vi "Init.vi"(8 "error in (no error)":errorcluster, 10 "ID":string, 11 "Deck in":refnum<class "Deck.lvclass">) -> (0 "error out":errorcluster, 3 "Deck out":refnum<class "Deck.lvclass">)   [LabVIEW 2019, in "Deck.lvclass"]
uses:
  Deck.lvclass
  State.ctl
  Packed Libraries/Audio Processing.lvlibp/Value Cluster.ctl
  Packed Libraries/Audio Processing.lvlibp/Value Properties.ctl
  Libraries/Track Info/Track Info.ctl
  Deck.lvclass/Deck.ctl
  Packed Libraries/Globals.lvlibp/Constants.vi
  Packed Libraries/Audio Processing.lvlibp
  Packed Libraries/Messaging.lvlibp
  Packed Libraries/Globals.lvlibp
  Libraries/Track Info/Track Info.lvlib
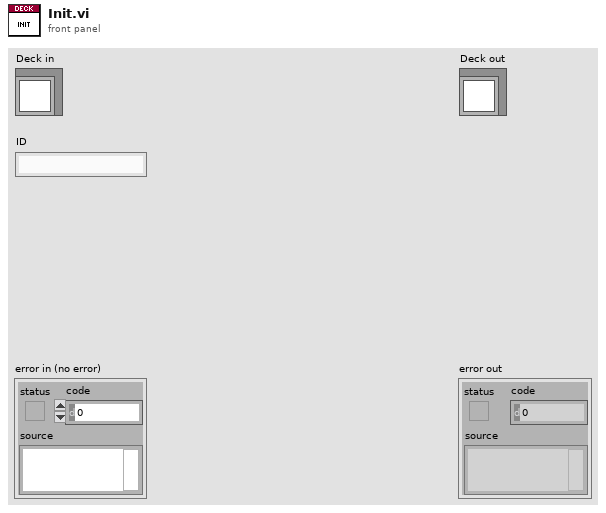
[diagram p1: front panel]
types:
  T1 = typedef "Track Info.lvlib/Track Info.ctl" = cluster{"Path":path, "Length (Samples)":i32, "Channels":i32, "Sample Rate (Hz)":i32, "BPM":dbl, "Cue Points (Samples)":i32[]}
  T2 = typedef "Audio Processing.lvlibp/Value Cluster.ctl" = cluster{"Value":dbl, "Properties":T3}
  T3 = typedef "Audio Processing.lvlibp/Value Properties.ctl" = cluster{"Lower":dbl, "Upper":dbl, "Default":dbl, "Increment":dbl}
  T4 = typedef "Deck.lvclass/State.ctl" = enum16{"No Track", "Loading", "Active", "Scratching", "Brake", "Backspin"}
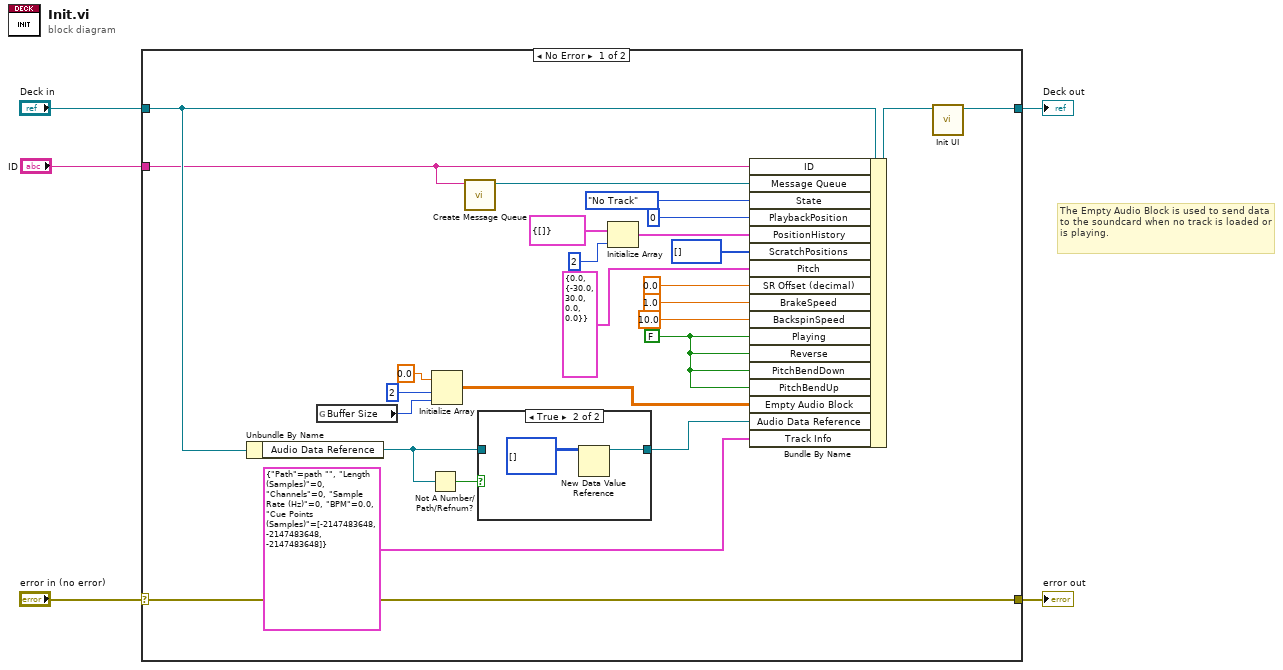
[diagram p0: block diagram]
diagram:
  # "The Empty Audio Block is used to send data to the soundcard when no track is loaded or is playing."
  n1 = case shown="No Error" "error in (no error)" {
    selector: "error in (no error)" -> [w30 w35]
    tunnel: [w30 w35] -> w4
    tunnel: [w6 w34] -> w2
    tunnel: "Deck in" -> [w25 w34]
    tunnel: "ID" -> [w12 _]
    frame No Error {
      w16 = FALSE ("PitchBendDown")
      n2 = Unbundle By Name(w25) -> ("Audio Data Reference"=w22:refnum<data-value>)
      n3 = global read "Constants.vi" "Buffer Size"() -> (w10:i32)
      n4 = Not A Number/Path/Refnum?(number/path/refnum=w22) -> (NaN/Path/Refnum?=w24:bool)
      n5 = Initialize Array(0.0, 2 ("dimension size"), w10) -> (w26:dbl[][])
      n6 = call "Create Message Queue.vi"("Queue Name"=w12) -> ("queue out"=w11:refnum<queue>)  [unwired: 9 in, 1 out]
      n7 = case shown="True" w24 {
        tunnel: [w31 w33] -> w23
        tunnel: w22 -> [w31 _]
        frame False {
        }
        frame True {
          n8 = New Data Value Reference(data value=i16[][] [] ("Audio Data")) -> (data value reference=w33:refnum<data-value>)  [unwired: 1 in, 1 out]
        }
      }
      n9 = Initialize Array(cluster{"Positions":i32[]} {"Positions"=[]} ("Cluster"), 2 ("dimension size")) -> (w18:cluster{"Positions":i32[]}[])
      n10 = Bundle By Name(cluster=w25, "ID"=w12, "Message Queue"=w11, "State"=State."No Track", "PlaybackPosition"=0 ("Playback Position (Samples)"), "PositionHistory"=w18, "ScratchPositions"=i32[] [], "Pitch"=T2 {"Value"=0.0, "Properties"={"Lower"=-30.0, "Upper"=30.0, "Default"=0.0, "Increment"=0.0}}, "SR Offset (decimal)"=0.0 ("Pitch Offset"), "BrakeSpeed"=1.0, "BackspinSpeed"=10.0, "Playing"=w16, "Reverse"=w16, "PitchBendDown"=w16, "PitchBendUp"=w16, "Empty Audio Block"=w26, "Audio Data Reference"=w23, "Track Info"=T1 {"Path"=path "", "Length (Samples)"=0, "Channels"=0, "Sample Rate (Hz)"=0, "BPM"=0.0, "Cue Points (Samples)"=[-2147483648, -2147483648, -2147483648]}) -> (w7:refnum<class "Deck.lvclass">)
      n11 = call "Init UI.vi"("Deck in"=w7) -> ("Deck out"=w6:refnum<class "Deck.lvclass">)  [unwired: 9 in, 1 out]
    }
    frame Error {
    }
  }
  "error out" <- w4
  "Deck out" <- w2
